vi "Arret RUN MODBUS EPC.vi"(0 "Port COM run 1 REG":refnum<visa-resource-name>, 1 "Adresse":u8, 2 "Choix consigne locale :":T1 items=["Consignes actuelles", "Mesures actuelles", "Valeur fixe pour tous les régulateurs"], 3 "error in":errorcluster, 4 "Valeur consigne":dbl) -> (5 "Consigne envoyée":dbl, 7 "error out":errorcluster)   [LabVIEW 2022 SP3]
uses:
  Enum/Commande Choix arret reg.ctl
  Variables globales/Variables glob EUROTHERM.vi
panel:
  out "Pt Mesure":sgl format="%.2f"
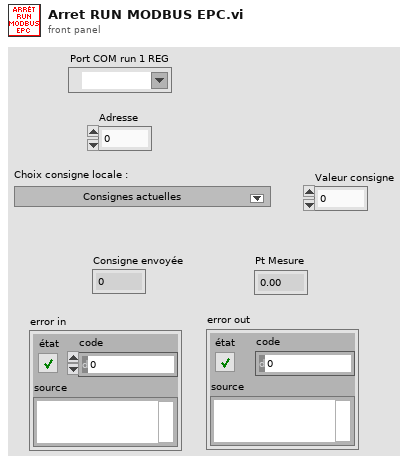
[diagram p1: front panel]
types:
  T1 = typedef "Commande Choix arret reg.ctl" = u16
  T2 = typedef "Semaphore RefNum" = refnum<k1>
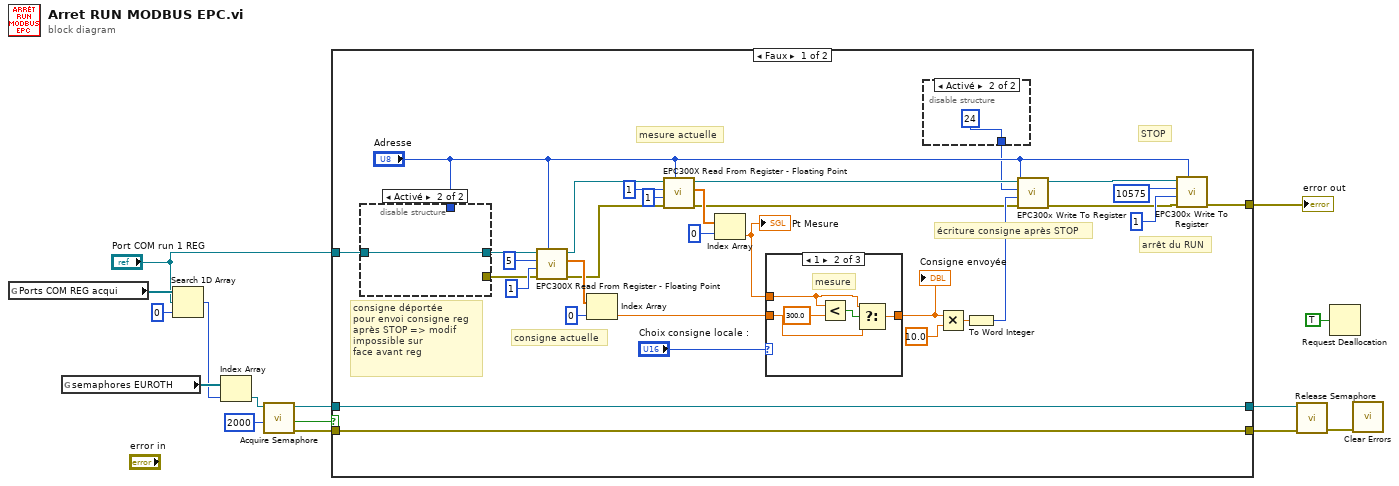
[diagram p0: block diagram]
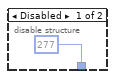
[diagram p2: hidden frame]
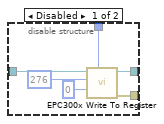
[diagram p3: hidden frame]
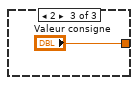
[diagram p5: hidden frame]
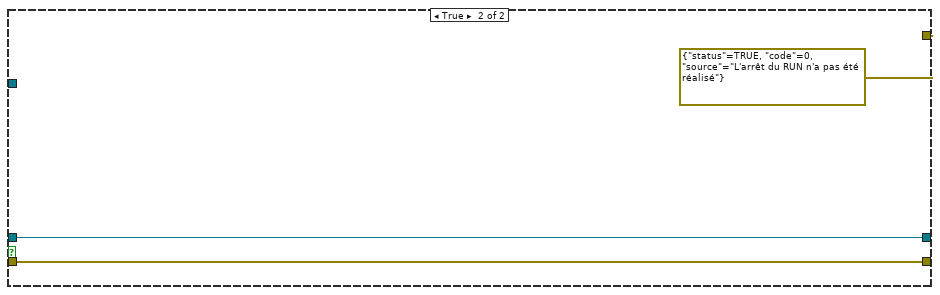
[diagram p6: hidden frame]
diagram:
  n1 = global read "Variables glob EUROTHERM.vi" "Ports COM REG acqui"() -> (w5:refnum<visa-resource-name>[])
  n2 = global read "Variables glob EUROTHERM.vi" "semaphores EUROTH"() -> (w7:T2[])
  n3 = Search 1D Array(1D array=w5, element="Port COM run 1 REG", start index (0)=0 ("indice de départ (0)")) -> (index of element=w2:i32)
  n4 = Index Array(array=w7, index=w2) -> (element=w6:T2)
  n5 = call <vilib>:"Acquire Semaphore.vi"("ms timeout (-1)"=2000, "semaphore"=w6) -> ("error out"=w12:errorcluster, "timed out"=w14:bool, "semaphore out"=w13:T2)  [unwired: 3 in]
  n6 = case shown="Faux" w14 {
    tunnel: w13 -> [w46 w65]
    tunnel: w12 -> [w45 w64]
    tunnel: [w46 w65] -> w10
    tunnel: [w45 w64] -> w9
    tunnel: "Port COM run 1 REG" -> [w37 _]
    tunnel: [w16 errorcluster {"status"=TRUE, "code"=0, "source"="L'arrêt du RUN n'a pas été réalisé"} ("error out")] -> w1
    frame False {
      # "écriture consigne après STOP"
      # "mesure actuelle"
      # "consigne déportée \npour envoi consigne reg\naprès STOP => modif \nimpossible sur\nface avant reg"
      # "STOP"
      # "arrêt du RUN"
      # "consigne actuelle"
      n7 = disable-structure shown="Activé" {
        disable-tunnel: w37 -> [w52 w55]
        disable-tunnel: [w51 w55] -> w36
        disable-tunnel: [w50 _] -> w35
        disable-tunnel: "Adresse" -> [w49 _]
        frame Disabled {
          n8 = call "EPC300x Write To Register.vi"("Unit Address (1)"=w49, "Data (0)"=i16 0, "Register Address (0)"=u16 276, "VISA session"=w52) -> ("error out"=w50:errorcluster, "dup VISA session"=w51:refnum<visa-resource-name>)  [unwired: 6 in]
        }
        frame Enabled {
        }
      }
      n9 = call "EPC300X Read From Register - Floating Point.vi"("Unit Address (1)"="Adresse", "error in (no error)"=w35, "Num Of Reg (1)"=u16 1, "Register Address (0)"=u16 5, "VISA session"=w36) -> ("error out"=w21:errorcluster, "Data (SGL)"=w43:sgl[], "dup VISA session"=w22:refnum<visa-resource-name>)  [unwired: 1 in, 3 out]
      n10 = Index Array(array=w43, index=0 ("indice")) -> (element=w40:sgl)
      n11 = call "EPC300X Read From Register - Floating Point.vi"("Unit Address (1)"="Adresse", "error in (no error)"=w21, "Num Of Reg (1)"=u16 1, "Register Address (0)"=u16 1, "VISA session"=w22) -> ("error out"=w27:errorcluster, "Data (SGL)"=w30:sgl[], "dup VISA session"=w28:refnum<visa-resource-name>)  [unwired: 1 in, 3 out]
      n12 = Index Array(array=w30, index=0 ("indice")) -> (element=w24:sgl)
      "Pt Mesure" <- w24
      n13 = case shown="1" "Choix consigne locale :" {
        tunnel: w40 -> [w56 w58 _]
        tunnel: [w56 w57 "Valeur consigne"] -> w23
        tunnel: w24 -> [_ w59 _]
        frame 0, Default {
          # "consigne"
        }
        frame 1 {
          # "mesure"
          n14 = Less?(x=w59, y=300.0) -> (x < y?=w60:bool)
          n15 = Select(t=w59, s=w60, f=w58) -> (s? t:f=w57:sgl)
        }
        frame 2 {
        }
      }
      "Consigne envoyée" <- w23
      n16 = disable-structure shown="Activé" {
        disable-tunnel: [u16 277 ("Register Address (0)") u16 24 ("Register Address (0)")] -> w17
        frame Disabled {
        }
        frame Enabled {
        }
      }
      n17 = Multiply(x=w23, y=sgl 10.0) -> (x*y=w34:dbl)
      n18 = To Word Integer(number=w34) -> (16bit integer=w33:i16)
      n19 = call "EPC300x Write To Register.vi"("Unit Address (1)"="Adresse", "error in (no error)"=w27, "Data (0)"=w33, "Register Address (0)"=w17, "VISA session"=w28) -> ("error out"=w19:errorcluster, "dup VISA session"=w20:refnum<visa-resource-name>)  [unwired: 5 in]
      n20 = call "EPC300x Write To Register.vi"("Unit Address (1)"="Adresse", "error in (no error)"=w19, "Data (0)"=i16 1, "Register Address (0)"=u16 10575, "VISA session"=w20) -> ("error out"=w16:errorcluster)  [unwired: 5 in, 1 out]
    }
    frame True {
    }
  }
  "error out" <- w1
  n21 = call <vilib>:"Release Semaphore.vi"("error in (no error)"=w9, "semaphore"=w10) -> ("error out"=w8:errorcluster)  [unwired: 4 in, 1 out]
  n22 = Request Deallocation(TRUE ("flag")) -> ()
  n23 = call <vilib>:"Clear Errors.vi"("error in (no error)"=w8) -> ()  [unwired: 5 in, 2 out]
